vi "RT_NetworkStreams.vi"() -> ()   [LabVIEW 2025]
uses:
  <vilib>/dex/Flush And Wait Empty Condition.ctl
panel:
  out "error out":errorcluster
  out "Waveform Graph":dbl[](graph)
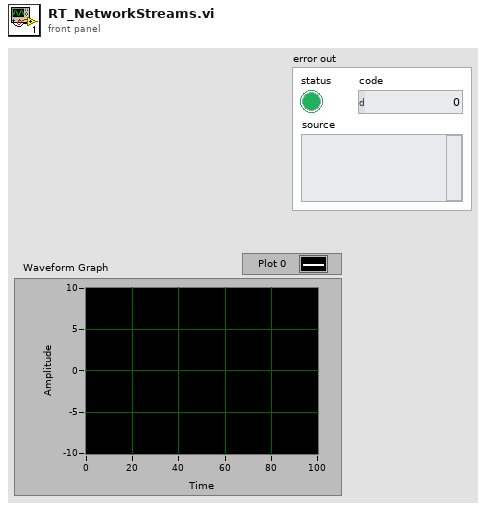
[diagram p1: front panel]
types:
  T1 = typedef "Flush And Wait Empty Condition.ctl" = u8
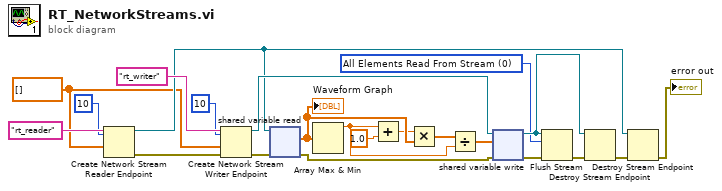
[diagram p0: block diagram]
diagram:
  w3 = dbl[] []
  w5 = T1 0 items=["All Elements Read From Stream", "All Elements Available for Reading"] ("wait condition")
  n1 = Create Network Stream Reader Endpoint(7:10 ("reader buffer size"), 9:w3, 11:"rt_reader" ("reader name")) -> (0:w22:errorcluster, 3:w6:refnum<k21>)  [unwired: 4 in]
  n2 = Create Network Stream Writer Endpoint(7:10 ("writer buffer size"), 8:w22, 9:w3, 11:"rt_writer" ("writer name")) -> (0:w21:errorcluster, 3:w12:refnum<k21>)  [unwired: 3 in]
  n3 = shared-variable-read(w6, w21) -> (w13:errorcluster, w18:dbl[])  [unwired: 1 in, 2 out]
  "Waveform Graph" <- w18
  n4 = Array Max & Min(array=w18) -> (max value=w14:dbl)  [unwired: 3 out]
  n5 = Add(x=w14, y=1.0) -> (x+y=w16:dbl)
  n6 = Multiply(x=w16, y=w18) -> (x*y=w15:dbl[])
  n7 = Divide(x=w15, y=w14) -> (x/y=w11:dbl[])
  n8 = shared-variable-write(w12, w13, w11) -> (w7:refnum<k21>, w10:errorcluster)  [unwired: 1 in, 1 out]
  n9 = Flush Stream(8:w10, 10:w5, 11:w7) -> (0:w9:errorcluster)  [unwired: 1 in, 2 out]
  n10 = Destroy Stream Endpoint(8:w9, 11:w7) -> (0:w8:errorcluster)
  n11 = Destroy Stream Endpoint(8:w8, 11:w6) -> (0:→"error out":errorcluster)
